vi "Check Labels.vi"(0 "Metric in":refnum<class "Metric.lvclass">, 11 "error in (no error)":errorcluster, 12 "Labels":map{string, string}(c390)) -> (4 "Samples":map{string, refnum<class "Sample.lvclass">}(c390), 6 "Valid Labels":bool, 8 "Label Values":string[](array[string]), 15 "error out":errorcluster)   [LabVIEW 2020, in "Metrics.lvlib" / "Metric.lvclass"]
uses:
  Metric.lvclass
  sample/Sample.lvclass
  Metric.lvclass/Metric.ctl
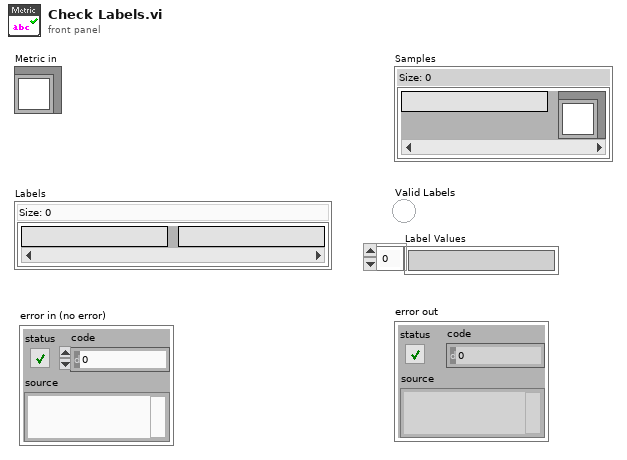
[diagram p1: front panel]
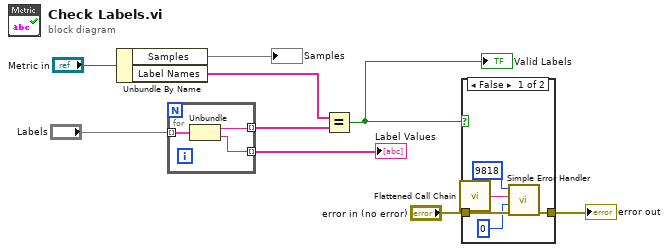
[diagram p0: block diagram]
diagram:
  n1 = Unbundle By Name("Metric in") -> ("Samples"=→"Samples":map{string, refnum<class "Sample.lvclass">}, "Label Names"=w6:string[])
  n2 = for {
    tunnel: "Labels" -> [w12] mode=indexing
    tunnel: [w11] -> w4 mode=indexing
    tunnel: [w10] -> w9 mode=indexing
    n3 = Unbundle(w12) -> ("labelname"=w11:string, "labelvalue"=w10:string)
  }
  "Label Values" <- w9
  n4 = Equal?(x=w6, y=w4) -> (x = y?=w3:bool)
  "Valid Labels" <- w3
  n5 = case shown="False" w3 {
    tunnel: "error in (no error)" -> [w17 w18]
    tunnel: [w13 w18] -> w1
    frame False {
      n6 = call "Flattened Call Chain.vi"() -> ("Flattened Call Chain"=w15:string)  [unwired: 5 in]
      n7 = call <vilib>:"Simple Error Handler.vi"("error code (no error:0)"=9818, "error source (\" \")"=w15, "type of dialog (OK msg:1)"=0 ("error code (no error:0)"), "error in (no error)"=w17) -> ("error out"=w13:errorcluster)  [unwired: 1 in, 4 out]
    }
    frame True {
    }
  }
  "error out" <- w1
